vi "Day 20-Process Image.vi"(10 "Lookup Array":bool[](array[boolean]), 11 "Image in":bool[][](array[boolean])) -> (3 "Image out":bool[][](array[boolean]))   [LabVIEW 2021]
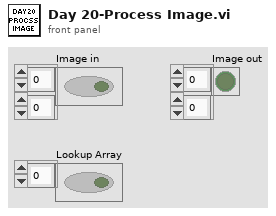
[diagram p1: front panel]
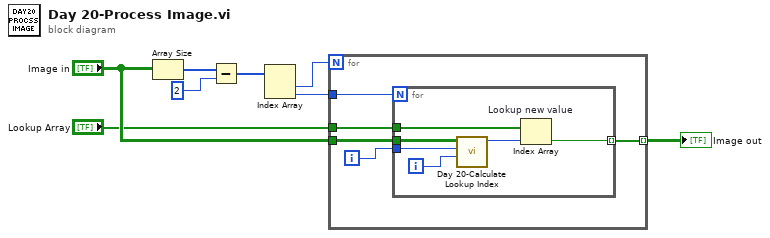
[diagram p0: block diagram]
diagram:
  n1 = Array Size(array="Image in") -> (size(s)=w7:i32[])
  n2 = Subtract(x=w7, y=2) -> (x-y=w3:i32[])
  n3 = Index Array(array=w3) -> (element #1=w2:i32, element #2=w1:i32)  [unwired: 2 in]
  n4 = for {
    N: w2 -> [_]
    tunnel: "Image in" -> [w12]
    tunnel: w1 -> [w11]
    tunnel: "Lookup Array" -> [w10]
    tunnel: [w9] -> w4 mode=indexing
    i -> [w13]
    n5 = for {
      N: w11 -> [_]
      tunnel: w12 -> [w18]
      tunnel: w10 -> [w17]
      tunnel: w13 -> [w15]
      tunnel: [w14] -> w9 mode=indexing
      i -> [w19]
      n6 = call "Day 20-Calculate Lookup Index.vi"("Left of Subgrid"=w19, "Top of Subgrid"=w15, "Image in"=w18) -> ("Lookup Index"=w16:u32)  [unwired: 8 in]
      n7 = Index Array "Lookup new value"(array=w17, index=w16) -> (element=w14:bool)
    }
  }
  "Image out" <- w4
